vi "Demo - dout.vi"() -> ()   [LabVIEW 2021]
uses:
  Dpin typedef.ctl
panel:
  in  "Value":bool
  in  "OUTPUT":bool
  out "error out":errorcluster
  in  "port":u32
  in  "Base URL":string
  in  "stop":bool
  in  "Digital pin":T1
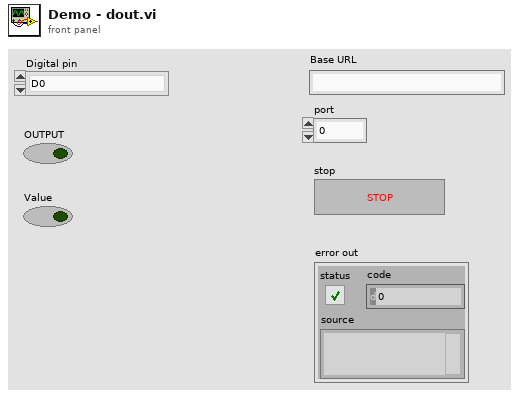
[diagram p1: front panel]
types:
  T1 = typedef "Dpin typedef.ctl" = enum16{"D0", "D1", "D2", "D3", "D4", "D5", "D6", "D7", "D8", "D9", "D10", "D11", "D12", "D13"}
  T2 = typedef "UNO Q Session.ctl" = cluster{"HTTP client":T3, "Base URL":string, "Connected":bool}
  T3 = typedef "LabVIEWHTTPClient.lvlib/ClientHandle.ctl" = refnum<k1>
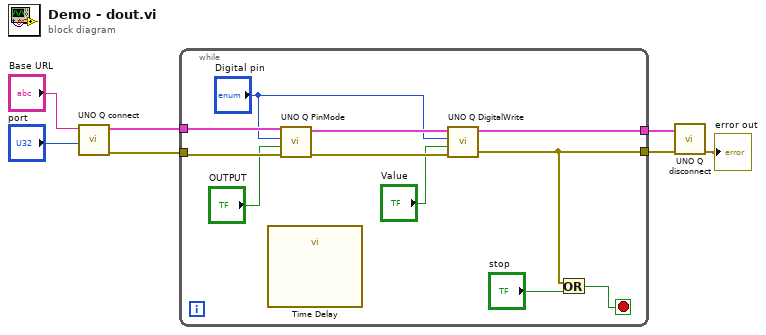
[diagram p0: block diagram]
diagram:
  n1 = call "UNO Q connect.vi"("port"="port", "Base URL"="Base URL") -> ("error out"=w4:errorcluster, "Session out"=w5:T2)  [unwired: 4 in]
  n2 = while {
    tunnel: w5 -> [w18]
    tunnel: w4 -> [w17]
    tunnel: [w13] -> w2
    tunnel: [w8] -> w1
    stop <- w9 stop-if-true
    n3 = call "Time Delay"() -> ()  [unwired: 11 in, 1 out]
    n4 = call "UNO Q PinMode.vi"("error in (no error)"=w17, "OUTPUT"="OUTPUT", "Digital pin"="Digital pin", "UNO Q Session in"=w18) -> ("error out"=w14:errorcluster, "UNO Q Session out"=w15:T2)  [unwired: 4 in, 2 out]
    n5 = call "UNO Q DigitalWrite.vi"("error in (no error)"=w14, "Value"="Value", "Digital pin"="Digital pin", "UNO Q Session in"=w15) -> ("error out"=w8:errorcluster, "UNO Q Session out"=w13:T2)  [unwired: 4 in, 2 out]
    n6 = Or(x=w8, y="stop") -> (x .or. y?=w9:bool)
  }
  n7 = call "UNO Q disconnect.vi"("error in (no error)"=w1, "UNO Q Session"=w2) -> ("error out"=→"error out":errorcluster)  [unwired: 9 in]
